vi "Read Entry.vi"(7 "Time Entry Store in":refnum<class "Time Entry Store-INI.lvclass">, 8 "error in (no error)":errorcluster, 10 "Start Time":timestamp, 11 "ID":string) -> (0 "error out":errorcluster, 2 "found?":bool, 3 "Time Entry":T1, 5 "Time Entry Store out":refnum<class "Time Entry Store-INI.lvclass">)   [LabVIEW 2024, in "Time Entry Store-INI.lvclass"]
doc: "Reads the time entry with the given ID from the month file of Start Time (UTC). found? is FALSE and the row is empty when it is not there.\n\nGenerated by: Claude"
uses:
  Time Entry Store-INI.lvclass
  Rows/Time Entry.ctl
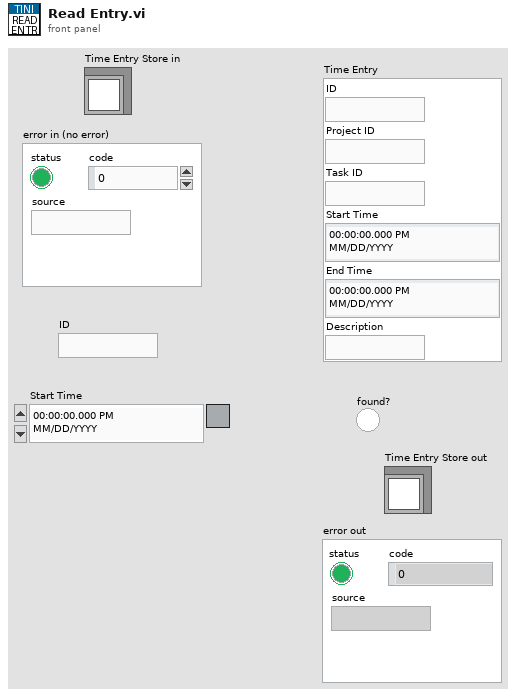
[diagram p1: front panel]
types:
  T1 = typedef "Time Entry.ctl" = cluster{"ID":string, "Project ID":string, "Task ID":string, "Start Time":timestamp, "End Time":timestamp, "Description":string}
  T2 = typedef "Time Entry List.ctl" = T1[]
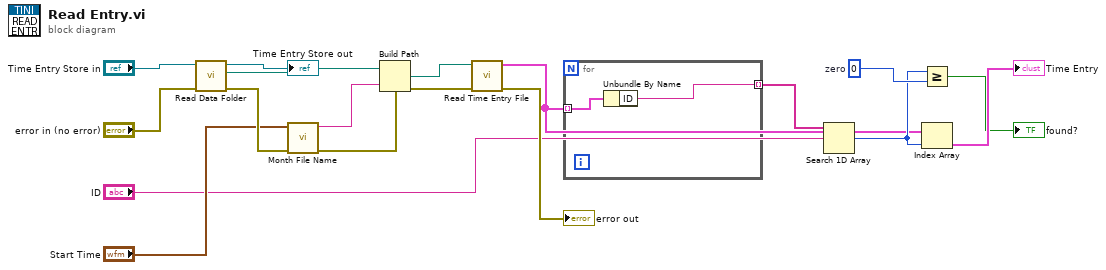
[diagram p0: block diagram]
diagram:
  w15 = 0  # zero
  n1 = call-dynamic "Read Data Folder.vi"("error in (no error)"="error in (no error)", "Time Entry Store-INI in"="Time Entry Store in") -> ("error out"=w5:errorcluster, "Data Folder"=w7:path, "Time Entry Store-INI out"=→"Time Entry Store out":refnum<class "Time Entry Store-INI.lvclass">)  [unwired: 7 in]
  n2 = call "Month File Name.vi"("error in (no error)"=w5, "Start Time"="Start Time") -> ("error out"=w9:errorcluster, "File Name"=w8:string)  [unwired: 8 in]
  n3 = Build Path(base path=w7, name or relative path=w8) -> (appended path=w10:path)
  n4 = call "Read Time Entry File.vi"("error in (no error)"=w9, "File Path"=w10) -> ("error out"=→"error out":errorcluster, "Time Entries"=w11:T2)  [unwired: 6 in, 2 out]
  n5 = for {
    tunnel: w11 -> [w18] mode=indexing
    tunnel: [w19] -> w13 mode=indexing
    n6 = Unbundle By Name(w18) -> ("ID"=w19:string)
  }
  n7 = Search 1D Array(1D array=w13, element="ID") -> (index of element=w14:i32)  [unwired: 1 in]
  n8 = Greater Or Equal?(x=w14, y=w15) -> (x >= y?=→"found?":bool)
  n9 = Index Array(array=w11, index=w14) -> (element=→"Time Entry":T1)
